vi "VIH Dialog - VI Terminals - Shortcut Menu Handler - Picture.vi"(4 "Class Name":string, 6 "Menu Tag":string, 8 "Tree Item Tag":string, 9 "MenuRef":refnum<k9>, 10 "Terminals Tree":refnum<vi>, 11 "Event Type":T1) -> (3 "States spec":string)   [LabVIEW 2014]
doc: "::: VI Helpeks :::\nCopyright (c) 2000-2026 Konstantin Shifershteyn. All rights reserved."
uses:
  <vilib>/event_ctls.llb/lveventtype.ctl
  <vilib>/Utility/miscctls.llb/LVNodeAndColumnTypeDef.ctl
  _VIH Support Library.llb/VIH Utility - MENU - Create Menu (String).vi
panel:
  # "VI Helpeks\nCopyright (c) 2012-2026 Konstantin Shifershteyn"
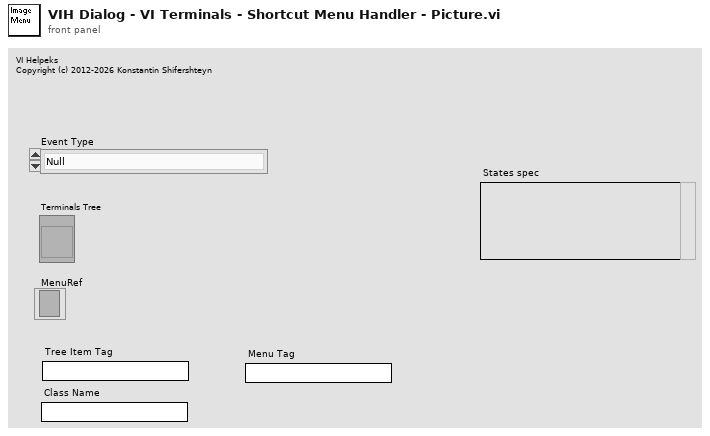
[diagram p1: front panel]
types:
  T1 = typedef "lveventtype.ctl" = enum32{"Null", "Timeout", "Annotation Menu Selection", "Annotation Menu Selection?", "App Instance Close", "App Instance Close?", "Autoscale Range Change", "Bookmark Info Change", "Cell Edit", "Cell Edit?", "Cursor Grab", "Cursor Grab?", "Cursor Menu Selection", "Cursor Menu Selection?", "Cursor Move", "Cursor Release", "Data Change", "Direction Change", "Display State Change", "Drag Ended", "Drag Enter", "Drag Leave", "Drag Over", "Drag Source Update", "Drag Starting", "Drag Starting?", "Drop", "Exec State Change", "Key Down", "Key Down?", "Key Repeat", "Key Repeat?", "Key Up", "Listbox Double Click", "Menu Activation?", "Menu Selection (App)", "Menu Selection? (App)", "Menu Selection (User)", "Mouse Down", "Mouse Down?", "Mouse Enter", "Mouse Leave", "Mouse Move", "Mouse Up", "Mouse Wheel", "NI Security User Change (App)", "Pane Size", "Panel Close", "Panel Close?", "Panel Resize", "Plot Attribute Change", "Scale Range Change", "Shortcut Menu Activation?", "Shortcut Menu Selection (App)", "Shortcut Menu Selection? (App)", "Shortcut Menu Selection (User)", "Tree Double Click", "Tree Drag", "Tree Drag?", "Tree Drop", "Tree Drop?", "Tree Item Close", "Tree Item Close?", "Tree Item Open", "Tree Item Open?", "User Event", "Value Change"}
  T2 = typedef "LVNodeAndColumnTypeDef.ctl" = cluster{"Node":string, "Column":i32}
  T3 = typedef "VIH Project Tree Typedef - Tree Refnum.ctl" = refnum<vi>
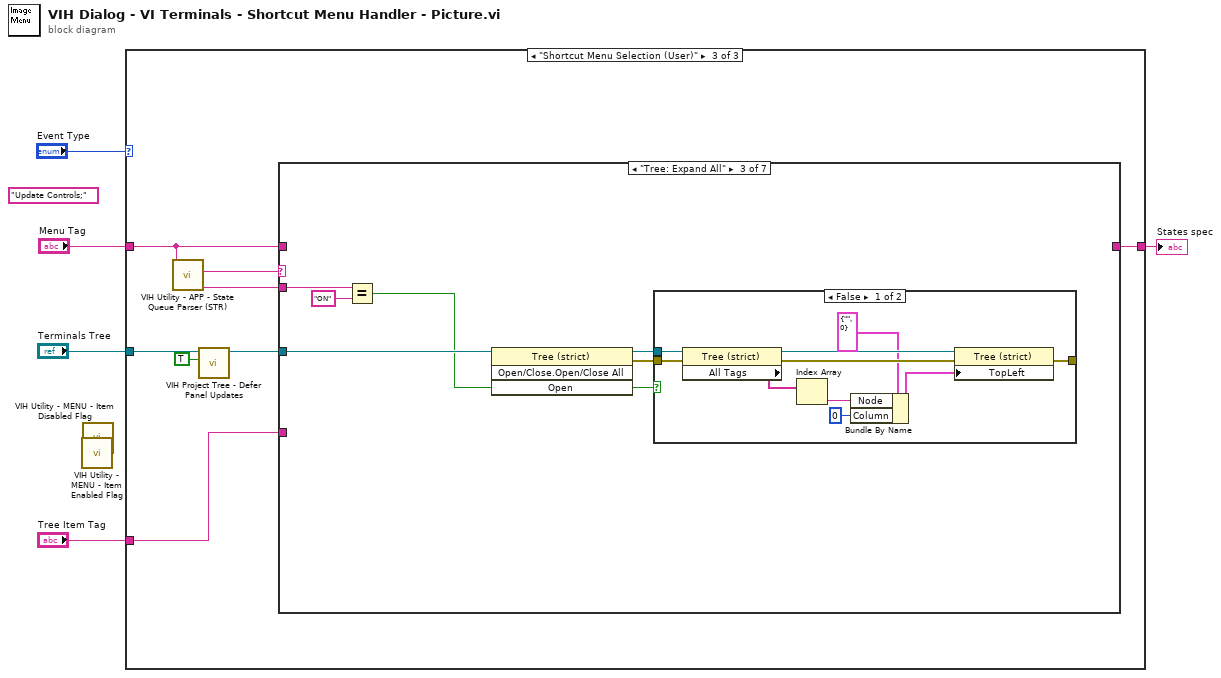
[diagram p0: block diagram]
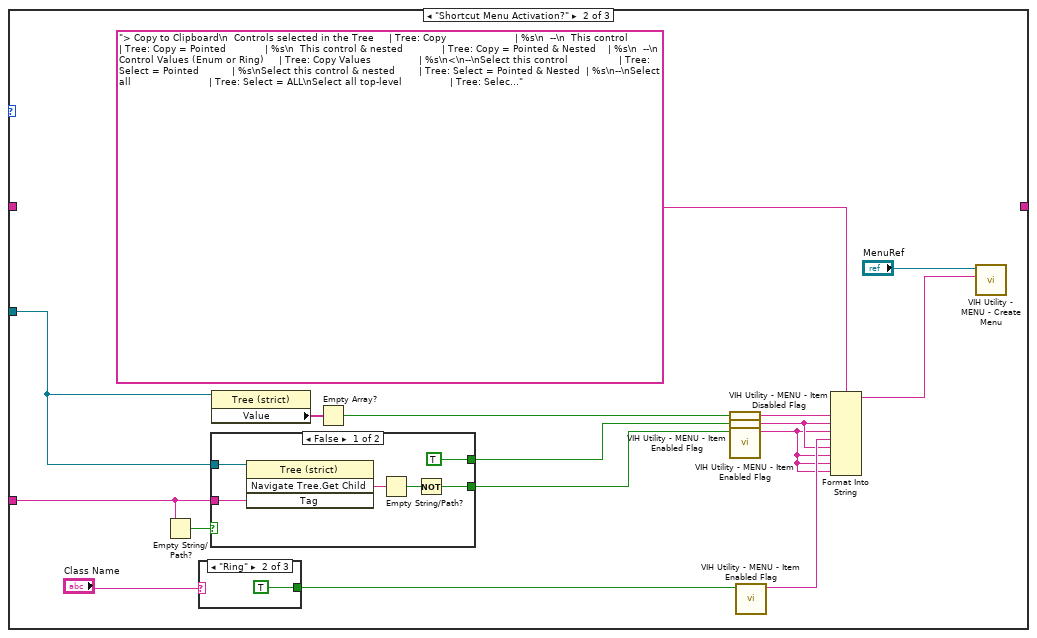
[diagram p3: hidden frame]
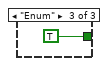
[diagram p5: hidden frame]
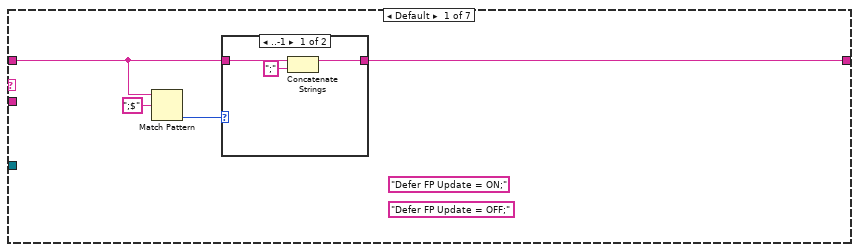
[diagram p7: hidden frame]
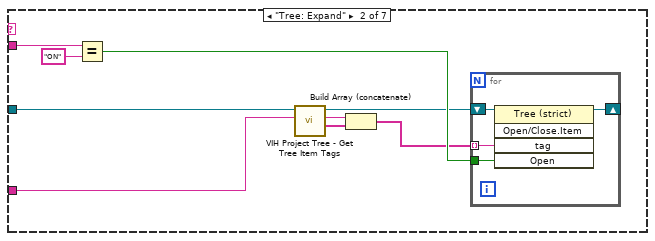
[diagram p9: hidden frame]
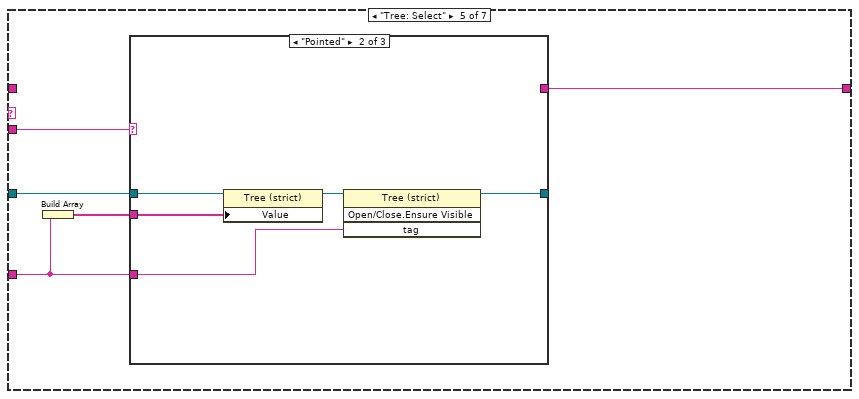
[diagram p12: hidden frame]
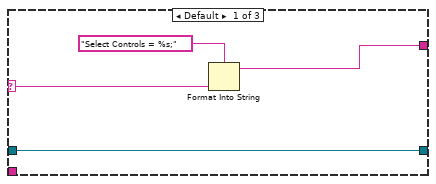
[diagram p13: hidden frame]
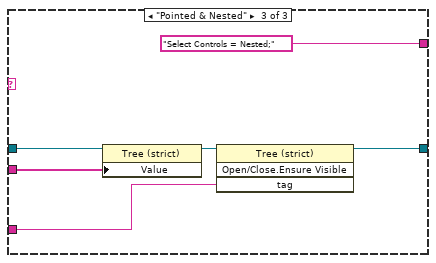
[diagram p14: hidden frame]
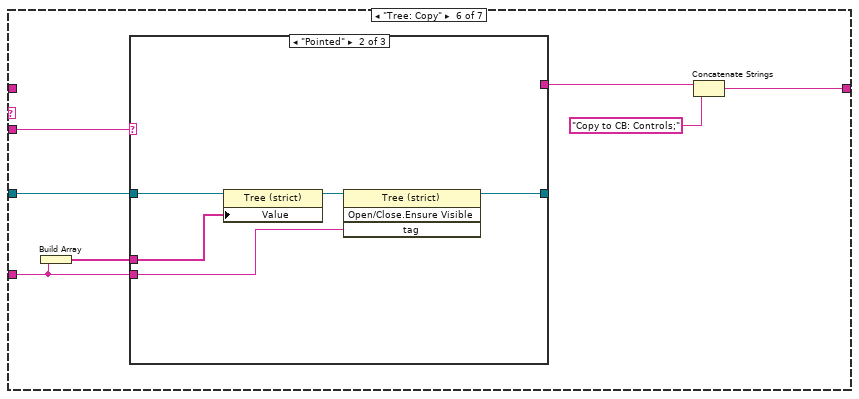
[diagram p15: hidden frame]
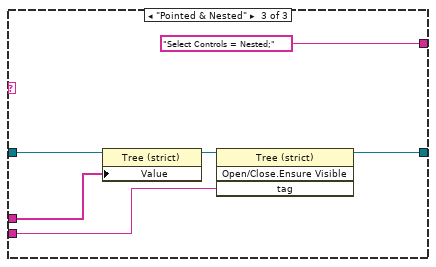
[diagram p17: hidden frame]
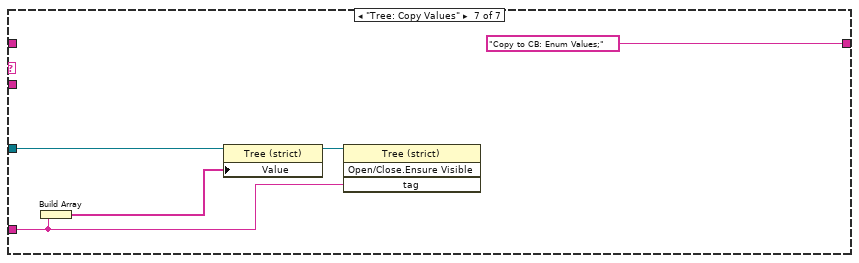
[diagram p18: hidden frame]
diagram:
  (unwired) "Update Controls;" ("Menu Tag")
  n1 = call "VIH Utility - MENU - Item Enabled Flag.vi"() -> ()  [unwired: 11 in, 1 out]
  n2 = call "VIH Utility - MENU - Item Disabled Flag.vi"() -> ()  [unwired: 11 in, 1 out]
  n3 = case shown="\"Shortcut Menu Selection (User)\"" "Event Type" {
    tunnel: "Terminals Tree" -> [_ w14 w31]
    tunnel: [_ _ w35] -> w3
    tunnel: "Menu Tag" -> [_ _ w36]
    tunnel: "Tree Item Tag" -> [_ w16 w33]
    frame Default {
    }
    frame "Shortcut Menu Activation?" {
      n4 = Empty String/Path?(string/path=w16) -> (empty?=w17:bool)
      n5 = case shown="\"Ring\"" "Class Name" {
        tunnel: [_ TRUE TRUE] -> w6
        frame Default {
        }
        frame "Ring" {
        }
        frame "Enum" {
        }
      }
      n6 = case shown="False" w17 {
        tunnel: [w27 _] -> w18
        tunnel: w14 -> [w26 _]
        tunnel: w16 -> [w25 _]
        tunnel: [TRUE _] -> w15
        frame False {
          n7 = invoke class="Tree (strict)" method="Navigate Tree.Get Child"(reference=w26, "Tag"=w25) -> ("Navigate Tree:Get Child"=w29:string)  [unwired: 2 in, 3 out]
          n8 = Empty String/Path?(string/path=w29) -> (empty?=w28:bool)
          n9 = Not(x=w28) -> (.not. x?=w27:bool)
        }
        frame True {
        }
      }
      n10 = property class="Tree (strict)"(reference=w14) -> ("Value"=w13:string[])  [unwired: 1 in, 2 out]
      n11 = Empty Array?(array=w13) -> (empty?=w12:bool)
      n12 = call "VIH Utility - MENU - Item Disabled Flag.vi"("Disable?"=w12) -> ("Disable flag"=w11:string)  [unwired: 10 in]
      n13 = call "VIH Utility - MENU - Item Enabled Flag.vi"("Enable?"=w15) -> ("Disable flag"=w9:string)  [unwired: 10 in]
      n14 = call "VIH Utility - MENU - Item Enabled Flag.vi"("Enable?"=w18) -> ("Disable flag"=w8:string)  [unwired: 10 in]
      n15 = call "VIH Utility - MENU - Item Enabled Flag.vi"("Enable?"=w6) -> ("Disable flag"=w10:string)  [unwired: 10 in]
      n16 = Format Into String(format string="> Copy to Clipboard\n  Controls selected in the Tree     | Tree: Copy                       | %s\n  --\n  This control                      | Tree: Copy = Pointed             | %s\n  This control & nested             | Tree: Copy = Pointed & Nested    | %s\n  --\n  Control Values (Enum or Ring)     | Tree: Copy Values                | %s\n<\n--\nSelect this control                 | Tree: Select = Pointed           | %s\nSelect this control & nested        | Tree: Select = Pointed & Nested  | %s\n--\nSelect all                          | Tree: Select = ALL\nSelect all top-level                | Tree: Select = Top-Level\nSelect all except error clusters    | Tree: Select = No Error\n// Select error clusters               | Tree: Select = Error\nSelect Enum & Ring controls         | Tree: Select = Enum & Ring\n--\n> Expand/Collapse Tree\n  Expand all                          | Tree: Expand All = ON\n  Collapse all                        | Tree: Expand All = OFF\n  --\n  Expand nested                       | Tree: Expand = ON                | %s\n  Collapse nested                     | Tree: Expand = OFF               | %s\n<", w11, w9, w8, w10, w9, w8, w8, w8) -> (resulting string=w19:string)  [unwired: 2 in, 1 out]
      n17 = call-poly "VIH Utility - MENU - Create Menu.vi"("Menu Description"=w19, "menu"="MenuRef") -> ()  [unwired: 8 in, 2 out]
    }
    frame "Shortcut Menu Selection (User)" {
      n18 = call "VIH Utility - APP - State Queue Parser (STR).vi"("input queue"=w36) -> ("state parameters"=w34:string, "state"=w37:string)  [unwired: 5 in, 2 out]
      n19 = call "VIH Project Tree - Defer Panel Updates.vi"("Defer Panel Updates (F)"=TRUE, "Project Tree"=w31) -> ("dup Project Tree"=w30:T3)  [unwired: 7 in, 2 out]
      n20 = case shown="\"Tree: Expand All\"" w37 {
        tunnel: [w38 _ _ _ w78 w98 "Copy to CB: Enum Values;"] -> w35
        tunnel: w36 -> [w39 _ _ _ _ _ _]
        tunnel: w30 -> [_ w46 w62 _ w76 w96 w115]
        tunnel: w33 -> [_ w54 _ _ w77 w99 w118]
        tunnel: w34 -> [_ w53 w64 _ w80 w102 _]
        frame Default {
          (unwired) "Defer FP Update = OFF;"
          (unwired) "Defer FP Update = ON;"
          n21 = Match Pattern(string=w39, regular expression=";$") -> (offset past match=w40:i32)  [unwired: 1 in, 3 out]
          n22 = case shown="..-1" w40 {
            tunnel: w39 -> [w44 w45]
            tunnel: [w43 w45] -> w38
            frame ..-1 {
              n23 = Concatenate Strings(w44, ";" ("string")) -> (w43:string)
            }
            frame 0.. {
            }
          }
        }
        frame "Tree: Expand" {
          n24 = Equal?(x=w53, y="ON") -> (x = y?=w51:bool)
          n25 = call "VIH Project Tree - Get Tree Item Tags.vi"("Parent Item Tag"=w54, "Project Tree"=w46) -> ("Child Item Tags"=w48:string[], "dup Parent Item Tag"=w49:string, "dup Project Tree"=w47:T3)  [unwired: 6 in, 1 out]
          n26 = Build Array (concatenate)(w49, w48) -> (w50:string[])
          n27 = for {
            tunnel: w50 -> [w57] mode=indexing
            tunnel: w51 -> [w56]
            shift-right: [w55] -> _
            shift-left: w47 -> [w58]
            n28 = invoke class="Tree (strict)" method="Open/Close.Item"(reference=w58, "tag"=w57, "Open"=w56) -> (reference out=w55:T3)  [unwired: 2 in, 4 out]
          }
        }
        frame "Tree: Expand All" {
          n29 = Equal?(x=w64, y="ON") -> (x = y?=w59:bool)
          n30 = invoke class="Tree (strict)" method="Open/Close.Open/Close All"(reference=w62, "Open"=w59) -> (reference out=w61:T3, error out=w60:errorcluster)  [unwired: 2 in, 2 out]
          n31 = case shown="False" w59 {
            tunnel: [w71 w75] -> _
            tunnel: w60 -> [w69 w75]
            tunnel: w61 -> [w68 _]
            frame False {
              n32 = property class="Tree (strict)"(reference=w68, error in=w69) -> (reference out=w67:T3, error out=w70:errorcluster, "All Tags"=w74:string[])
              n33 = Index Array(array=w74) -> (element=w73:string)  [unwired: 1 in]
              n34 = Bundle By Name(cluster=T2 {"Node"="", "Column"=0} ("Top Left Visible Cell"), "Node"=w73, "Column"=0) -> (w65:T2)
              n35 = property class="Tree (strict)"(reference=w67, error in=w70, "TopLeft"=w65) -> (error out=w71:errorcluster)  [unwired: 1 out]
            }
            frame True {
            }
          }
        }
        frame "----------------------------- 1" {
        }
        frame "Tree: Select" {
          n36 = Build Array(w77) -> (w79:string[])
          n37 = case shown="\"Pointed\"" w80 {
            selector: w80 -> [w84 _ _]
            tunnel: w76 -> [w81 w89 w95]
            tunnel: w79 -> [_ w88 w94]
            tunnel: [w82 _ "Select Controls = Nested;"] -> w78
            tunnel: w77 -> [_ w86 w91]
            tunnel: [w81 w85 w90] -> _
            frame Default {
              n38 = Format Into String(format string="Select Controls = %s;", w84) -> (resulting string=w82:string)  [unwired: 2 in, 1 out]
            }
            frame "Pointed" {
              n39 = property on="Property Node" class="Tree (strict)"(reference=w89, "Value"=w88) -> (reference out=w87:T3)  [unwired: 1 in, 1 out]
              n40 = invoke class="Tree (strict)" method="Open/Close.Ensure Visible"(reference=w87, "tag"=w86) -> (reference out=w85:T3)  [unwired: 2 in, 3 out]
            }
            frame "Pointed & Nested" {
              n41 = property on="Property Node" class="Tree (strict)"(reference=w95, "Value"=w94) -> (reference out=w92:T3)  [unwired: 1 in, 1 out]
              n42 = invoke class="Tree (strict)" method="Open/Close.Ensure Visible"(reference=w92, "tag"=w91) -> (reference out=w90:T3)  [unwired: 2 in, 3 out]
            }
          }
        }
        frame "Tree: Copy" {
          n43 = Build Array(w99) -> (w101:string[])
          n44 = case shown="\"Pointed\"" w102 {
            tunnel: w96 -> [w103 w108 w114]
            tunnel: w101 -> [_ w107 w113]
            tunnel: [_ _ "Select Controls = Nested;"] -> w100
            tunnel: w99 -> [_ w105 w110]
            tunnel: [w103 w104 w109] -> _
            frame Default {
            }
            frame "Pointed" {
              n45 = property on="Property Node" class="Tree (strict)"(reference=w108, "Value"=w107) -> (reference out=w106:T3)  [unwired: 1 in, 1 out]
              n46 = invoke class="Tree (strict)" method="Open/Close.Ensure Visible"(reference=w106, "tag"=w105) -> (reference out=w104:T3)  [unwired: 2 in, 3 out]
            }
            frame "Pointed & Nested" {
              n47 = property on="Property Node" class="Tree (strict)"(reference=w114, "Value"=w113) -> (reference out=w111:T3)  [unwired: 1 in, 1 out]
              n48 = invoke class="Tree (strict)" method="Open/Close.Ensure Visible"(reference=w111, "tag"=w110) -> (reference out=w109:T3)  [unwired: 2 in, 3 out]
            }
          }
          n49 = Concatenate Strings(w100, "Copy to CB: Controls;") -> (w98:string)
        }
        frame "Tree: Copy Values" {
          n50 = Build Array(w118) -> (w119:string[])
          n51 = property on="Property Node" class="Tree (strict)"(reference=w115, "Value"=w119) -> (reference out=w117:T3)  [unwired: 1 in, 1 out]
          n52 = invoke class="Tree (strict)" method="Open/Close.Ensure Visible"(reference=w117, "tag"=w118) -> ()  [unwired: 2 in, 4 out]
        }
      }
    }
  }
  "States spec" <- w3
